vi "Coerce Size.vi"(3 "Min Size":cluster{"Width":i32, "Height":i32}, 4 "Size":cluster{"Width":i32, "Height":i32}, 5 "Max Size":cluster{"Width":i32, "Height":i32}={"Width"=1024, "Height"=768}) -> (1 "Coerced Size":cluster{"Width":i32, "Height":i32})   [LabVIEW 2012]
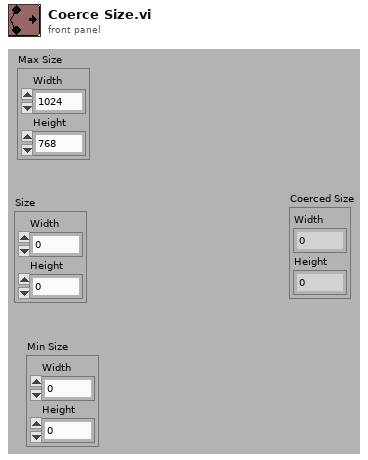
[diagram p1: front panel]
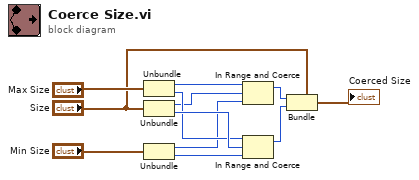
[diagram p0: block diagram]
diagram:
  n1 = Unbundle("Max Size") -> ("Width"=w9:i32, "Height"=w8:i32)
  n2 = Unbundle("Size") -> ("Width"=w7:i32, "Height"=w10:i32)
  n3 = Unbundle("Min Size") -> ("Width"=w2:i32, "Height"=w1:i32)
  n4 = In Range and Coerce(upper limit=w9, x=w7, lower limit=w2) -> (coerced(x)=w12:i32)  [unwired: 1 out]
  n5 = In Range and Coerce(upper limit=w8, x=w10, lower limit=w1) -> (coerced(x)=w11:i32)  [unwired: 1 out]
  n6 = Bundle(cluster="Size", "Width"=w12, "Height"=w11) -> (→"Coerced Size":cluster{"Width":i32, "Height":i32})
